vi "LTE select Device.vi"(8 "error in (no error)":errorcluster caption="에러 입력(에러 없음)", 11 "Instrument Manager 입력":refnum<class "Instrument Manager.lvclass">) -> (0 "error out":errorcluster caption="에러 출력", 3 "Instrument Manager 출력":refnum<class "Instrument Manager.lvclass">)   [LabVIEW 2023, in "Instrument Manager.lvclass"]
uses:
  Instrument Manager.lvclass
  Instrument Manager.lvclass/Instrument Manager.ctl
  Module/ANRITSU Call Box/Interface Class/Anritsu Call Box.lvclass
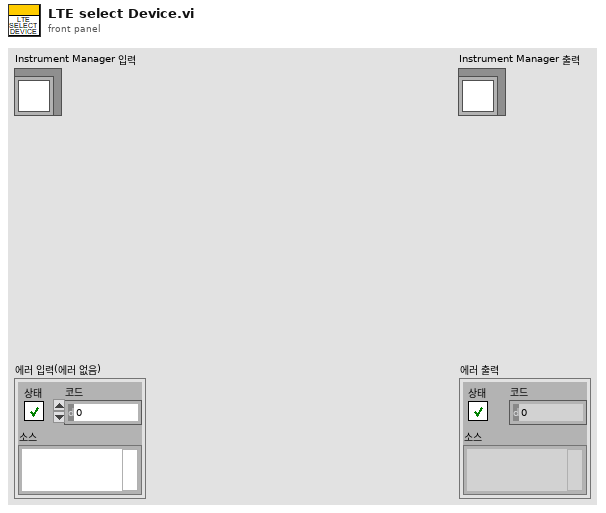
[diagram p1: front panel]
types:
  T1 = cluster{"Anritsu Call Box":refnum<class "Anritsu Call Box.lvclass">, "Spectrum Analyzer":refnum<class "Interface_Spectrum.lvclass">, "RF Switch Box":refnum<class "RF Filter Box.lvclass">, "Turn Table":refnum<class "Interface - Turn Table.lvclass">, "Mast":refnum<class "Interface - Mast.lvclass">, "3D Controller":refnum<class "Interface_3D Controller.lvclass">}
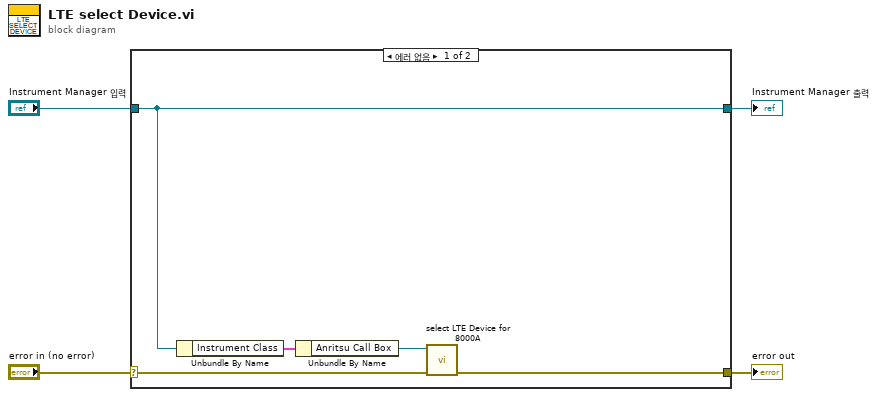
[diagram p0: block diagram]
diagram:
  n1 = case shown="에러 없음" "error in (no error)" {
    selector: "error in (no error)" -> [w9 w11]
    tunnel: [w5 w11] -> w3
    tunnel: [w8 w10] -> w1
    tunnel: "Instrument Manager 입력" -> [w8 w10]
    frame No Error {
      n2 = Unbundle By Name(w8) -> ("Instrument Class"=w7:T1)
      n3 = Unbundle By Name(w7) -> ("Anritsu Call Box"=w6:refnum<class "Anritsu Call Box.lvclass">)
      n4 = call-dynamic "select LTE Device for 8000A.vi"("error in (no error)"=w9, "Anritsu Call Box in"=w6) -> ("error out"=w5:errorcluster)  [unwired: 8 in, 1 out]
    }
    frame Error {
    }
  }
  "error out" <- w3
  "Instrument Manager 출력" <- w1
